vi "D_W_FMemBMPPath.vi"(8 "error in (no error)":errorcluster, 9 "slotNo":u32, 10 "BMP file path":path, 11 "bID":u8) -> (0 "error out":errorcluster, 3 "bID":u8, 4 "TorF":i32)   [LabVIEW 2018]
uses:
  hpkSLMdaLV.dll
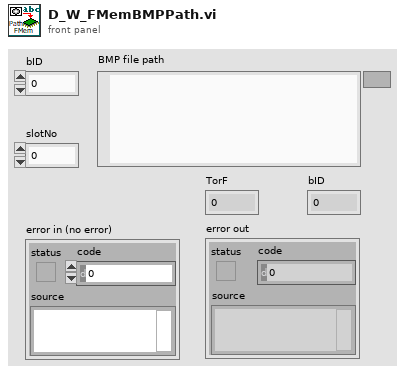
[diagram p1: front panel]
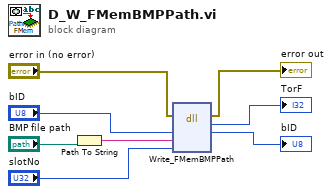
[diagram p0: block diagram]
diagram:
  n1 = Path To String(path="BMP file path") -> (string=w6:string)
  n2 = dll-call lib="PTH2ﾅunc \\\\K45292-FS\\Data\n荳ｭ遐猫COSpost譛晉ｨｲ\n08_LabVIEW!00_繝ｩ繝懊ン繝･繝ｼ繝励Ο繧ｰ繝ｩ繝LabVIEW2018 LCOS_DriverV3.0_Hardware_ControlUSB_Multi-ControlHardwareControl_LVhpkSLMdaLV.dll" fn="Write_FMemBMPPath"(error in="error in (no error)", "bID"="bID", "path"=w6, "slotNo"="slotNo") -> (error out=→"error out":errorcluster, "返り値タイプ"=→"TorF":i32, "bID"=→"bID":u8)  [unwired: 4 in, 1 out]
